vi "DSS-Tests-paths.vi"() -> (2 "repo root":path, 3 "tests folder":path)   [LabVIEW 2020, in "DSS-Tests.lvlib"]
doc: "Returns the folder of the DSS test suite (the folder of this VI) and the repository root three folders above it, so every test builds its data paths without an absolute path."
uses:
  DSS-Tests.lvlib
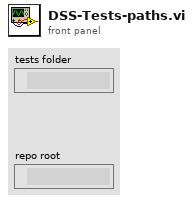
[diagram p1: front panel]
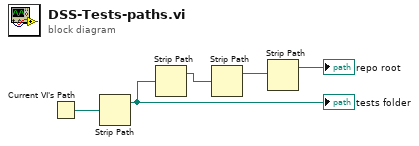
[diagram p0: block diagram]
diagram:
  n1 = Current VI's Path() -> (path=w1:path)
  n2 = Strip Path(path=w1) -> (stripped path=w2:path)  [unwired: 1 out]
  "tests folder" <- w2
  n3 = Strip Path(path=w2) -> (stripped path=w3:path)  [unwired: 1 out]
  n4 = Strip Path(path=w3) -> (stripped path=w4:path)  [unwired: 1 out]
  n5 = Strip Path(path=w4) -> (stripped path=→"repo root":path)  [unwired: 1 out]
